vi "RDC-permittivity-handle_all.vi"(7 "basic data(open, short, water, ...)":T1[](array[typedef]), 11 "Data Array":T1[](array[typedef])) -> (3 "Common Format out":T1[](array[typedef]))   [LabVIEW 2020, in "RDC-Reflection_Data_Computation.lvlib"]
doc: "Computes the permittivity of every Common Format cluster in Data Array with each calculation type of RDC-permittivity_collection, using the basic data."
uses:
  RDC-Reflection_Data_Computation.lvlib
  Reflector/RFH-common_data_format.ctl
  RDC-perm_calc_type.ctl
  Reflector/RFH-Reflection_File_Handler.lvlib
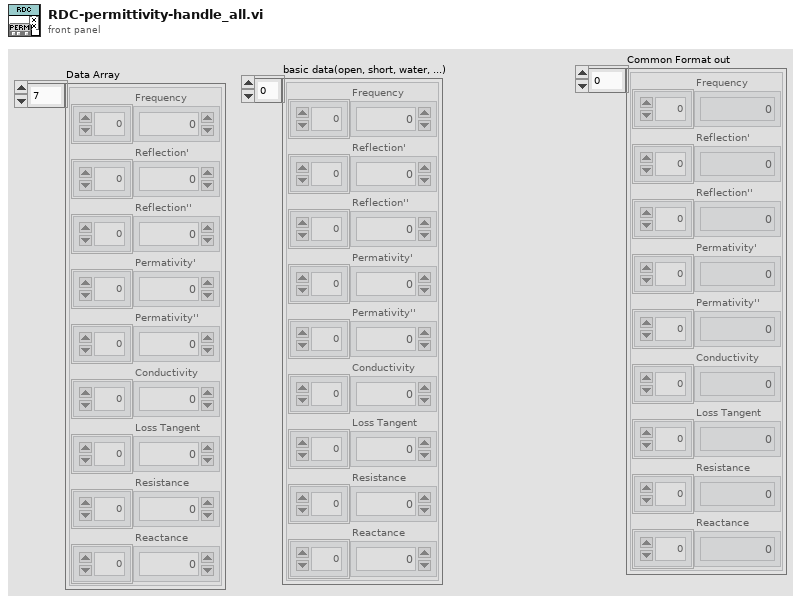
[diagram p1: front panel]
types:
  T1 = typedef "RFH-Reflection_File_Handler.lvlib/RFH-common_data_format.ctl" = cluster{"Frequency":dbl[], "Reflection'":dbl[], "Reflection''":dbl[], "Permativity'":dbl[], "Permativity''":dbl[], "Conductivity":dbl[], "Loss Tangent":dbl[], "Resistance":dbl[], "Reactance":dbl[]}
  T2 = typedef "RDC-Reflection_Data_Computation.lvlib/RDC-perm_calc_type.ctl" = enum16{"Basic", "Capacative", "Advance", "Bilinear", "Size"}
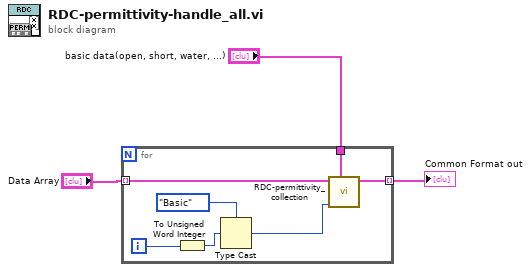
[diagram p0: block diagram]
diagram:
  n1 = for {
    tunnel: "basic data(open, short, water, ...)" -> [w10]
    tunnel: "Data Array" -> [w9] mode=indexing
    tunnel: [w8] -> w1 mode=indexing
    i -> [w7]
    n2 = To Unsigned Word Integer(number=w7) -> (unsigned 16bit integer=w6:u16)
    n3 = Type Cast(type=RDC-perm_calc_type."Basic" ("Perm calc type"), x=w6) -> (*(type *) &x=w4:T2)
    n4 = call "RDC-permittivity_collection.vi"("basic data(open, short, water)"=w10, "Perm calc type"=w4, "Common Format"=w9) -> ("Common Format 2"=w8:T1)  [unwired: 8 in]
  }
  "Common Format out" <- w1
